vi "VIH HelpGen - Build Log Handler.vi"(6 "cmd (nop)":T1(ring), 8 "error in":errorcluster, 9 "Files #":cluster{"Files total":i32, "Files ptoc":i32}, 10 "Out File Path":path, 11 "Src File Path":path) -> (0 "error out":errorcluster, 1 "HTML Paths":path[](array[path]), 2 "errors":i32, 3 "log file path":path, 4 "CHM Path":path)   [LabVIEW 2014]
doc: "::: VI Helpeks :::\nCopyright (c) 2000-2026 Konstantin Shifershteyn. All rights reserved."
panel:
  # "VI Helpeks\nCopyright (c) 2012-2026 Konstantin Shifershteyn"
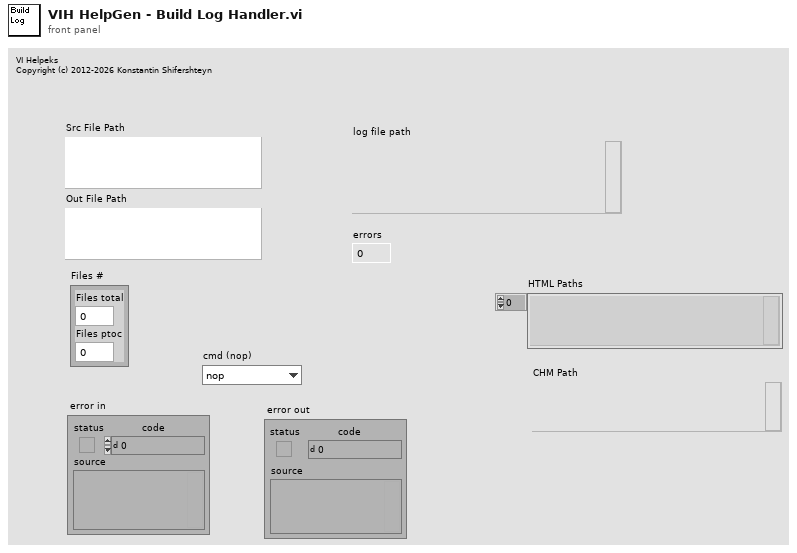
[diagram p1: front panel]
types:
  T1 = enum16{"nop", "Start", "Stop", "Run-prep", "Run-VI", "Run-Menu"}
  T2 = cluster{"Src Paths":path[], "Errors":errorcluster[], "Out Paths":path[]}
  T3 = cluster{"Project file":path, "Build Log file":path, "Start TS":timestamp, "Finish TS":timestamp, "Files total":i32, "Files proc":i32, "Errors":i32}
  T4 = enum16{"nop", "Init", "Run-HHP", "Run-CHM", "Run-INFO"}
  T5 = cluster{"HHP Built":bool, "HHP file":path, "HHP Error":errorcluster, "CHM Built":bool, "CHM file":path, "CHM Error":errorcluster, "INFO Built":bool, "Info file":path, "INFO Error":errorcluster}
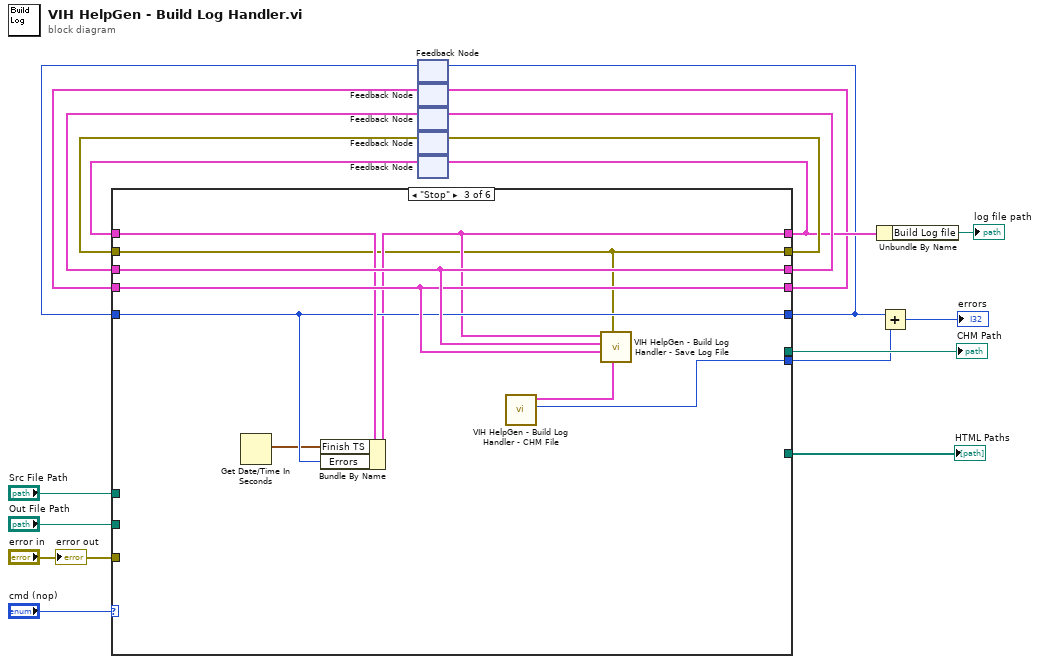
[diagram p0: block diagram]
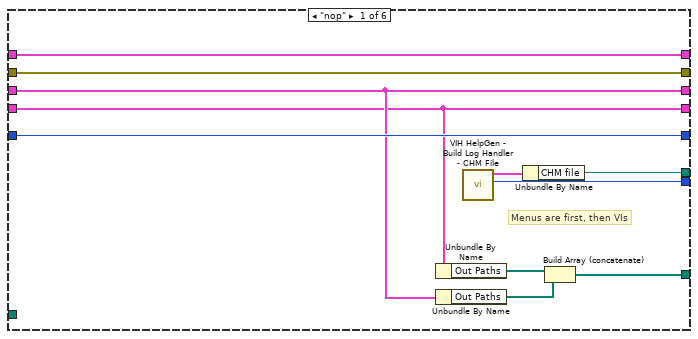
[diagram p2: hidden frame]
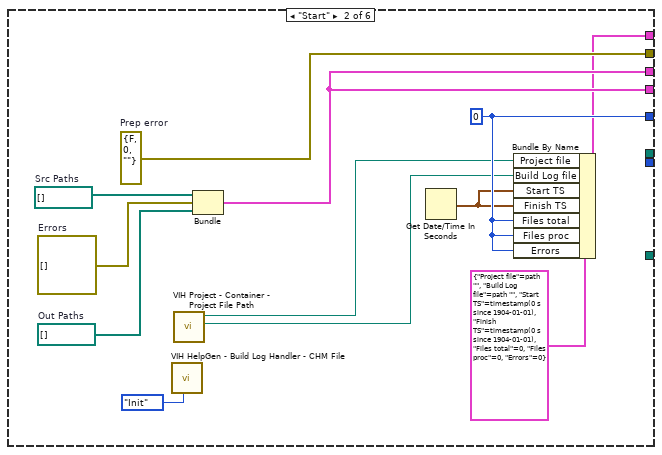
[diagram p3: hidden frame]
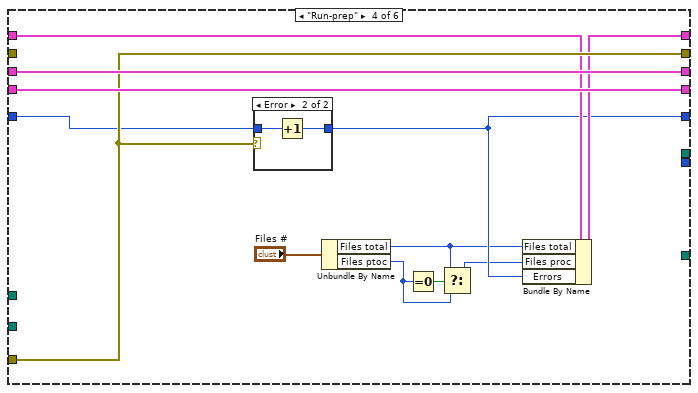
[diagram p4: hidden frame]
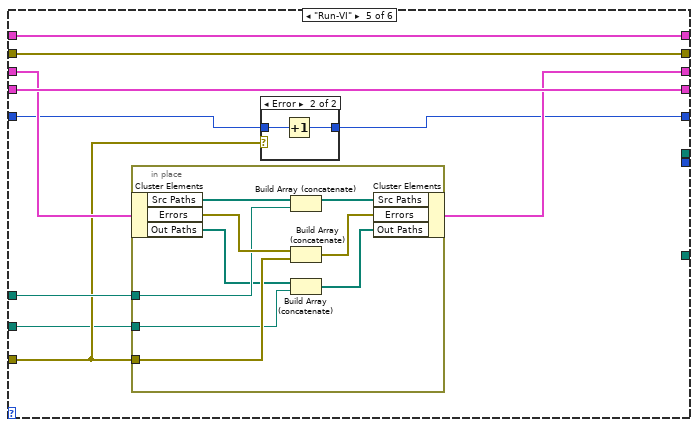
[diagram p6: hidden frame]
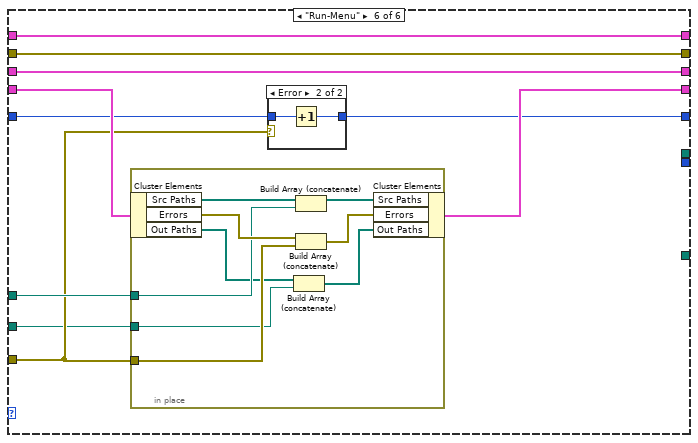
[diagram p8: hidden frame]
diagram:
  n1 = feedback #1() -> (w10:i32)  [unwired: 1 in]
  n2 = feedback #2() -> (w12:T2)  [unwired: 1 in]
  n3 = feedback #3() -> (w13:T2)  [unwired: 1 in]
  n4 = feedback #4() -> (w15:errorcluster)  [unwired: 1 in]
  n5 = feedback #5() -> (w17:T3)  [unwired: 1 in]
  n6 = case shown="\"Stop\"" "cmd (nop)" {
    tunnel: [w30 w34 w46 w58 w76 w98] -> w9
    tunnel: "Src File Path" -> [_ _ _ _ w73 w96]
    tunnel: w17 -> [w30 _ w49 w59 w76 w98]
    tunnel: [w29 w40 w45 w61 w74 w97] -> w16
    tunnel: w15 -> [w29 _ w45 _ w74 w97]
    tunnel: [w27 w39 w51 w63 w71 w95] -> w14
    tunnel: [w26 w39 w50 w62 w75 w93] -> w6
    tunnel: w13 -> [w27 _ w51 w63 w72 w95]
    tunnel: w12 -> [w26 _ w50 w62 w75 w94]
    tunnel: "error in" -> [_ _ _ w61 w69 w91]
    tunnel: [w28 w37 w48 w57 w68 w90] -> w3
    tunnel: w10 -> [w28 _ w48 w60 w70 w92]
    tunnel: "Out File Path" -> [_ _ _ _ w67 w89]
    tunnel: [w23 _ _ _ _ _] -> w5
    tunnel: [w21 _ _ _ _ _] -> w4
    tunnel: [w20 _ w43 _ _ _] -> w1
    frame "nop" {
      # "Menus are first, then VIs"
      n7 = Unbundle By Name(w26) -> ("Out Paths"=w25:path[])
      n8 = Unbundle By Name(w27) -> ("Out Paths"=w24:path[])
      n9 = call "VIH HelpGen - Build Log Handler - CHM File.vi"() -> ("errors"=w20:i32, "CHM status"=w22:T5)  [unwired: 9 in, 1 out]
      n10 = Unbundle By Name(w22) -> ("CHM file"=w21:path)
      n11 = Build Array (concatenate)(w25, w24) -> (w23:path[])
    }
    frame "Start" {
      w32 = path[] []  # Out Paths
      w37 = 0
      w40 = errorcluster {"status"=FALSE, "code"=0, "source"=""}  # Prep error
      w41 = errorcluster[] []  # Errors
      w42 = path[] []  # Src Paths
      n12 = call "VIH HelpGen - Build Log Handler - CHM File.vi"("cmd (nop)"=T4."Init") -> ()  [unwired: 8 in, 3 out]
      n13 = call "VIH Project - Container - Project File Path.vi"() -> ("Project Build Log File"=w33:path, "Project File Path"=w36:path)  [unwired: 9 in, 1 out]
      n14 = Bundle("Src Paths"=w42, "Errors"=w41, "Out Paths"=w32) -> (w39:T2)  [unwired: 1 in]
      n15 = Get Date/Time In Seconds() -> (seconds since 1Jan1904=w35:timestamp)
      n16 = Bundle By Name(cluster=T3 {"Project file"=path "", "Build Log file"=path "", "Start TS"=timestamp(0 s since 1904-01-01), "Finish TS"=timestamp(0 s since 1904-01-01), "Files total"=0, "Files proc"=0, "Errors"=0} ("Cluster"), "Project file"=w36, "Build Log file"=w33, "Start TS"=w35, "Finish TS"=w35, "Files total"=w37, "Files proc"=w37, "Errors"=w37) -> (w34:T3)
    }
    frame "Stop" {
      n17 = Get Date/Time In Seconds() -> (seconds since 1Jan1904=w47:timestamp)
      n18 = Bundle By Name(cluster=w49, "Finish TS"=w47, "Errors"=w48) -> (w46:T3)
      n19 = call "VIH HelpGen - Build Log Handler - CHM File.vi"() -> ("errors"=w43:i32, "CHM status"=w44:T5)  [unwired: 9 in, 1 out]
      n20 = call "VIH HelpGen - Build Log Handler - Save Log File.vi"("CHM status"=w44, "preparation error"=w45, "Menu Help status"=w50, "VI Help status"=w51, "Status"=w46) -> ()  [unwired: 6 in, 1 out]
    }
    frame "Run-prep" {
      n21 = case shown="Error" w61 {
        tunnel: w60 -> [w64 w66]
        tunnel: [w64 w65] -> w57
        frame No Error {
        }
        frame Error {
          n22 = Increment(x=w66) -> (x+1=w65:i32)
        }
      }
      n23 = Unbundle By Name("Files #") -> ("Files total"=w54:i32, "Files ptoc"=w53:i32)
      n24 = Equal To 0?(x=w53) -> (x = 0?=w55:bool)
      n25 = Select(t=w54, s=w55, f=w53) -> (s? t:f=w52:i32)
      n26 = Bundle By Name(cluster=w59, "Files total"=w54, "Files proc"=w52, "Errors"=w57) -> (w58:T3)
    }
    frame "Run-VI" {
      n27 = in-place {
        in-place-border: w73 -> [w84]
        in-place-border: w69 -> [w83]
        in-place-border: w67 -> [w81]
        n28 = in-place-cluster #6(w72) -> ("Src Paths"=w88:path[], "Errors"=w86:errorcluster[], "Out Paths"=w82:path[])
        n29 = Build Array (concatenate)(w88, w84) -> (w87:path[])
        n30 = Build Array (concatenate)(w86, w83) -> (w85:errorcluster[])
        n31 = Build Array (concatenate)(w82, w81) -> (w80:path[])
        n32 = in-place-cluster #6("Src Paths"=w87, "Errors"=w85, "Out Paths"=w80) -> (w71:T2)
      }
      n33 = case shown="Error" w69 {
        tunnel: w70 -> [w77 w79]
        tunnel: [w77 w78] -> w68
        frame No Error {
        }
        frame Error {
          n34 = Increment(x=w79) -> (x+1=w78:i32)
        }
      }
    }
    frame "Run-Menu" {
      n35 = in-place {
        in-place-border: w96 -> [w106]
        in-place-border: w91 -> [w105]
        in-place-border: w89 -> [w103]
        n36 = in-place-cluster #7(w94) -> ("Src Paths"=w110:path[], "Errors"=w108:errorcluster[], "Out Paths"=w104:path[])
        n37 = Build Array (concatenate)(w104, w103) -> (w102:path[])
        n38 = Build Array (concatenate)(w110, w106) -> (w109:path[])
        n39 = Build Array (concatenate)(w108, w105) -> (w107:errorcluster[])
        n40 = in-place-cluster #7("Src Paths"=w109, "Errors"=w107, "Out Paths"=w102) -> (w93:T2)
      }
      n41 = case shown="Error" w91 {
        tunnel: w92 -> [w99 w101]
        tunnel: [w99 w100] -> w90
        frame No Error {
        }
        frame Error {
          n42 = Increment(x=w101) -> (x+1=w100:i32)
        }
      }
    }
  }
  "HTML Paths" <- w5
  "CHM Path" <- w4
  n43 = feedback-in #1(w3) -> ()
  n44 = feedback-in #2(w6) -> ()
  n45 = feedback-in #3(w14) -> ()
  n46 = feedback-in #4(w16) -> ()
  n47 = feedback-in #5(w9) -> ()
  n48 = Unbundle By Name(w9) -> ("Build Log file"=→"log file path":path)
  n49 = Add(x=w3, y=w1) -> (x+y=→"errors":i32)
  "error out" <- "error in"
